vi "laser_constant_current_output.vi"(9 "Laser Active Ref":refnum<vi>, 10 "Stop Ref":refnum<vi>, 11 "Current Ref":refnum<vi>) -> ()   [LabVIEW 2025, in "tSNIP.lvlib"]
uses:
  tSNIP.lvlib
panel:
  in  "VISA resource name":refnum<visa-resource-name>="Laser_Controller"
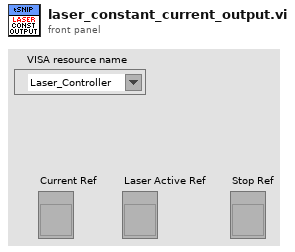
[diagram p1: front panel]
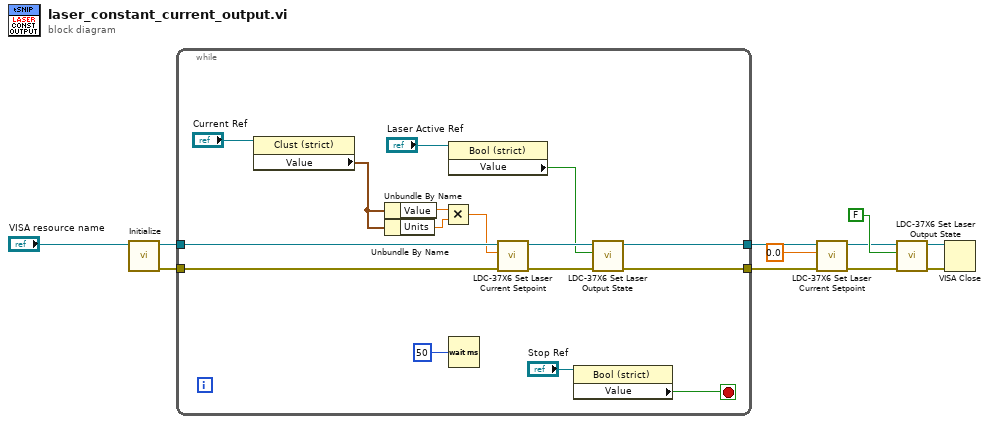
[diagram p0: block diagram]
diagram:
  n1 = call "Initialize.vi"("VISA resource name"="VISA resource name") -> ("error out"=w9:errorcluster, "VISA resource name out"=w10:refnum<visa-resource-name>)  [unwired: 9 in]
  n2 = while {
    tunnel: w10 -> [w25]
    tunnel: w9 -> [w26]
    tunnel: [w24] -> w8
    tunnel: [w23] -> w7
    stop <- w12 stop-if-true
    n3 = property class="Clust (strict)"(reference="Current Ref") -> ("Value"=w16:cluster{"Value":dbl, "Units":dbl})  [unwired: 1 in, 2 out]
    n4 = Unbundle By Name(w16) -> ("Value"=w20:dbl)
    n5 = Unbundle By Name(w16) -> ("Units"=w19:dbl)
    n6 = Multiply(x=w20, y=w19) -> (x*y=w18:dbl)
    n7 = property class="Bool (strict)"(reference="Laser Active Ref") -> ("Value"=w14:bool)  [unwired: 1 in, 2 out]
    n8 = Wait (ms)(milliseconds to wait=u32 50) -> ()  [unwired: 1 out]
    n9 = call <instrlib>:"LDC-37X6 Set Laser Current Setpoint.vi"("VISA resource name"=w25, "Laser Current Setpoint (A)"=w18, "error in"=w26) -> ("VISA resource name out"=w22:refnum<visa-resource-name>, "error out"=w21:errorcluster)  [unwired: 6 in]
    n10 = property class="Bool (strict)"(reference="Stop Ref") -> ("Value"=w12:bool)  [unwired: 1 in, 2 out]
    n11 = call <instrlib>:"LDC-37X6 Set Laser Output State.vi"("error in"=w21, "Laser Output Enable"=w14, "VISA resource name"=w22) -> ("error out"=w24:errorcluster, "VISA resource name out"=w23:refnum<visa-resource-name>)  [unwired: 7 in]
  }
  n12 = call <instrlib>:"LDC-37X6 Set Laser Current Setpoint.vi"("VISA resource name"=w7, "Laser Current Setpoint (A)"=0.0, "error in"=w8) -> ("VISA resource name out"=w3:refnum<visa-resource-name>, "error out"=w5:errorcluster)  [unwired: 6 in]
  n13 = call <instrlib>:"LDC-37X6 Set Laser Output State.vi"("error in"=w5, "Laser Output Enable"=FALSE, "VISA resource name"=w3) -> ("error out"=w1:errorcluster, "VISA resource name out"=w2:refnum<visa-resource-name>)  [unwired: 7 in]
  n14 = VISA Close(VISA resource name=w2, error in (no error)=w1) -> ()  [unwired: 1 out]
